vi "Test Generate Mock Class Creates lvclass File.vi"(8 "error in (no error)":errorcluster, 11 "Test Case In":refnum<class "_Mock Class Generator Test.lvclass">) -> (0 "error out":errorcluster, 3 "Test Case Out":refnum<class "_Mock Class Generator Test.lvclass">)   [LabVIEW 2020, in "_Mock Class Generator Test.lvclass"]
uses:
  _Mock Class Generator Test.lvclass
  C:/Program Files (x86)/National Instruments/LabVIEW 2020/vi.lib/Astemes/LUnit/Test Case.lvclass
  <vilib>/Astemes/LUnit/Test Case.lvclass/Test Case.ctl
  <vilib>/Astemes/LUnit/Append Fail Result.vi
  <vilib>/Astemes/LUnit/Append Pass Result.vi
  <vilib>/Astemes/LUnit/Run In UI.vi
  <vilib>/Utility/error.llb/Clear Errors.vi
  source/Scripting/Mock Class Generator/Mock Class Generator.lvclass
  <vilib>/Astemes/LUnit/Test Case.lvclass
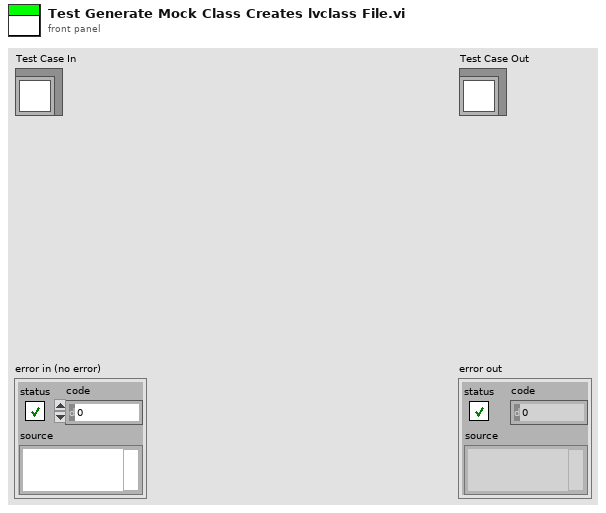
[diagram p1: front panel]
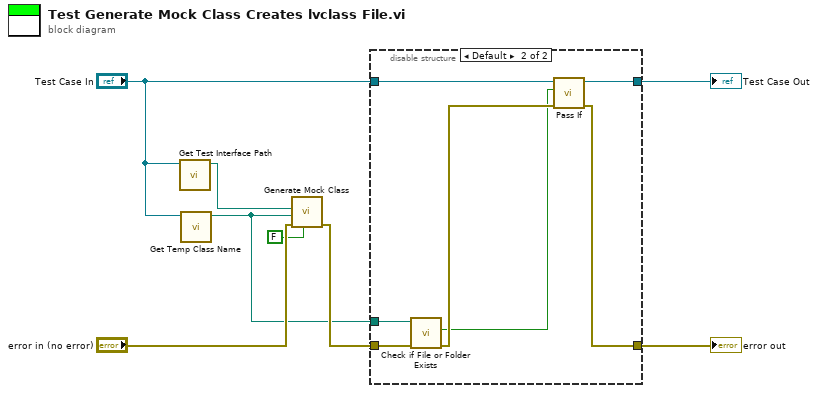
[diagram p0: block diagram]
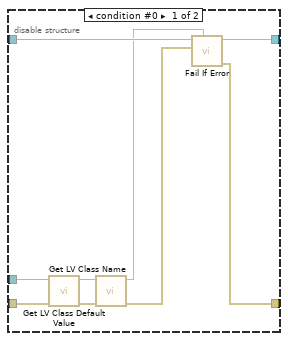
[diagram p2: hidden frame]
diagram:
  n1 = call "Get Test Interface Path.vi"("Mock Class Generator Test in"="Test Case In") -> ("Test Class Path"=w6:path)  [unwired: 10 in]
  n2 = call "Get Temp Class Name.vi"("Mock Class Generator Test in"="Test Case In") -> ("Test Class Path"=w2:path)  [unwired: 10 in]
  n3 = call "Generate Mock Class.vi"("Add to lvproj?"=FALSE, "error in (no error)"="error in (no error)", "Destination Class Path"=w2, "Source Class Path"=w6) -> ("error out"=w3:errorcluster)  [unwired: 6 in, 1 out]
  n4 = disable-structure shown="Default" {
    disable-tunnel: [w17 w24] -> w8
    disable-tunnel: [w16 w23] -> w7
    disable-tunnel: "Test Case In" -> [w15 w22]
    disable-tunnel: w3 -> [w14 w21]
    disable-tunnel: w2 -> [w12 w20]
    frame condition #0 {
      n5 = call <vilib>:"Get LV Class Default Value.vi"("error in (no error)"=w14, "class path"=w12) -> ("error out"=w13:errorcluster, "object"=w11:refnum<class>)  [unwired: 8 in]
      n6 = call <vilib>:"Get LV Class Name.vi"("error in (no error)"=w13, "object"=w11) -> ("error out"=w9:errorcluster, "class name"=w10:string)  [unwired: 8 in]
      n7 = call <vilib>:"Fail If Error.vi"("Description"=w10, "Assert error"=w9, "LUnit Test Case In"=w15) -> ("error out"=w16:errorcluster, "LUnit Test Case Out"=w17:refnum<class "_Mock Class Generator Test.lvclass">)  [unwired: 7 in]
    }
    frame condition #1 (active) {
      n8 = call <vilib>:"Check if File or Folder Exists.vi"("error in (no error)"=w21, "path"=w20) -> ("error out"=w19:errorcluster, "file or folder exists?"=w18:bool)  [unwired: 7 in, 1 out]
      n9 = call <vilib>:"Pass If.vi"("error in (no error)"=w19, "Pass?"=w18, "LUnit Test Case In"=w22) -> ("error out"=w23:errorcluster, "LUnit Test Case Out"=w24:refnum<class "_Mock Class Generator Test.lvclass">)  [unwired: 7 in]
    }
  }
  "error out" <- w7
  "Test Case Out" <- w8
